vi "Obtain Request Events.vi"(8 "error in":errorcluster, 10 "Create New? (F)":bool, 11 "Module ID":i32=-1) -> (0 "error out":errorcluster, 2 "Function Generator Request Events":T1)   [LabVIEW 2026, in "Function Generator.lvlib"]
doc: "This VI Obtains/Creates the Requests events that will be used for other modules to communicate with the module that owns this VI. These Requests events will be accessed only via Public API methods for this module.\n\n<b>NOTE</b>: The contents of this VI are automatically generated and modified by the <b>Tools > DQMH Consortium > DQMH</b> utilities. Consider using those utilities instead of making your own modifications to this VI.\n_____\nBased on DQMH Dev Tools: Project Template 7.1.2.1547."
uses:
  Function Generator.lvlib
  Request Events--cluster.ctl
  Stop Argument--cluster.ctl
  Show Panel Argument--cluster.ctl
  Hide Panel Argument--cluster.ctl
  Show Diagram Argument--cluster.ctl
  Get Module Execution Status Argument--cluster.ctl
  Set Signal Type Argument--cluster.ctl
  Set Signal Parameters Argument--cluster.ctl
  Start Argument--cluster.ctl
  Local Instance Request Events--cluster.ctl
  Wake Up HL Argument--cluster.ctl
  Stop FGEN Argument--cluster.ctl
  Local Instance Events SEQ/Local Instance Events SEQ.lvlib
panel:
  # "NOTE: The contents of this VI are automatically generated and modified by the Tools > DQMH Consortium > DQMH utilities. Consider using those utilities instead of making your own modifications to this VI."
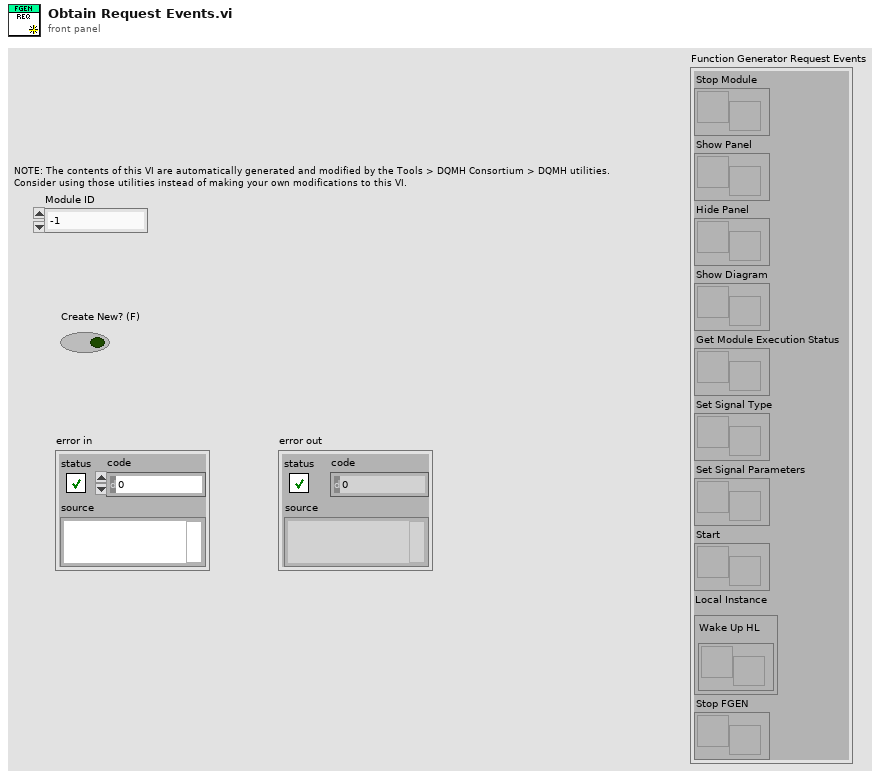
[diagram p1: front panel]
types:
  T1 = typedef "Function Generator.lvlib/Request Events--cluster.ctl" = cluster{"Stop Module":refnum<user-event>, "Show Panel":refnum<user-event>, "Hide Panel":refnum<user-event>, "Show Diagram":refnum<user-event>, "Get Module Execution Status":refnum<user-event>, "Set Signal Type":refnum<user-event>, "Set Signal Parameters":refnum<user-event>, "Start":refnum<user-event>, "Local Instance":T2, "Stop FGEN":refnum<user-event>}
  T2 = typedef "Function Generator.lvlib/Local Instance Request Events--cluster.ctl" = cluster{"Wake Up HL":refnum<user-event>}
  T3 = typedef "Function Generator.lvlib/Stop FGEN Argument--cluster.ctl" = cluster{"Module ID":i32, "Boolean":bool}
  T4 = typedef "Function Generator.lvlib/Start Argument--cluster.ctl" = cluster{"Module ID":i32, "Boolean":bool}
  T5 = typedef "Function Generator.lvlib/Set Signal Parameters Argument--cluster.ctl" = cluster{"Module ID":i32, "amplitude":dbl, "phase":dbl, "frequency":dbl, "offset":dbl}
  T6 = typedef "Function Generator.lvlib/Set Signal Type Argument--cluster.ctl" = cluster{"Module ID":i32, "signal type":enum16{"Sine Wave", "Triangle Wave", "Square Wave", "Sawtooth Wave"}}
  T7 = typedef "Function Generator.lvlib/Get Module Execution Status Argument--cluster.ctl" = cluster{"Module ID":i32, "Running?":bool}
  T8 = typedef "Function Generator.lvlib/Show Diagram Argument--cluster.ctl" = cluster{"Module ID":i32, "Debug?":bool}
  T9 = typedef "Function Generator.lvlib/Show Panel Argument--cluster.ctl" = cluster{"Module ID":i32, "Show Panel?":bool}
  T10 = typedef "Function Generator.lvlib/Hide Panel Argument--cluster.ctl" = cluster{"Module ID":i32, "Hide Panel?":bool}
  T11 = typedef "Function Generator.lvlib/Stop Argument--cluster.ctl" = cluster{"Module ID":i32, "Origin":string, "Exit via Stop Module Req?":bool, "Wait for Module to stop?":bool}
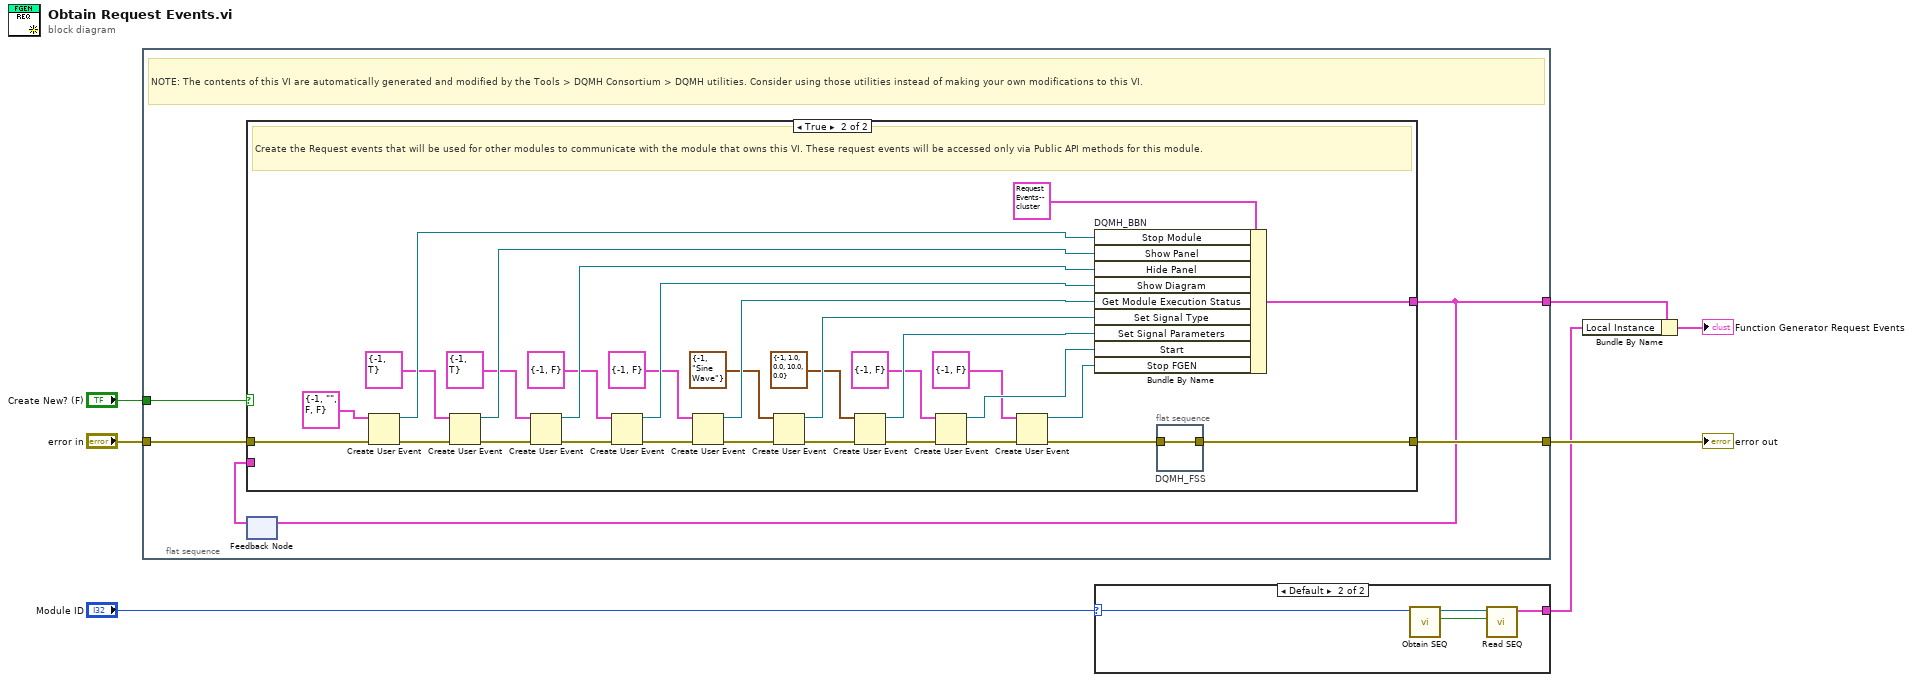
[diagram p0: block diagram]
diagram:
  n1 = flat-sequence {
    tunnel: [w12] -> w7
    tunnel: "error in" -> [w11]
    tunnel: [w9] -> w3
    tunnel: "Create New? (F)" -> [w8]
    frame #0 {
      # "NOTE: The contents of this VI are automatically generated and modified by the Tools > DQMH Consortium > DQMH utilities. Consider using those utilities instead of making your own modifications to this VI."
      n2 = feedback #1() -> (w10:T1)  [unwired: 1 in]
      n3 = case shown="True" w8 {
        tunnel: [w13 w33] -> w12
        tunnel: w11 -> [w13 w45]
        tunnel: [w14 w42] -> w9
        tunnel: w10 -> [w14 _]
        frame False {
        }
        frame True {
          # "Create the Request events that will be used for other modules to communicate with the module that owns this VI. These request events will be accessed only via Public API methods for this module."
          n4 = Create User Event(user event datatype=T11 {"Module ID"=-1, "Origin"="", "Exit via Stop Module Req?"=FALSE, "Wait for Module to stop?"=FALSE} ("Stop Argument"), error in=w45) -> (user event=w43:refnum<user-event>, error out=w40:errorcluster)
          n5 = Create User Event(user event datatype=T9 {"Module ID"=-1, "Show Panel?"=TRUE} ("Show Panel Argument"), error in=w40) -> (user event=w39:refnum<user-event>, error out=w37:errorcluster)
          n6 = Create User Event(user event datatype=T10 {"Module ID"=-1, "Hide Panel?"=TRUE} ("Hide Panel"), error in=w37) -> (user event=w36:refnum<user-event>, error out=w35:errorcluster)
          n7 = Create User Event(user event datatype=T8 {"Module ID"=-1, "Debug?"=FALSE} ("Show Diagram Argument"), error in=w35) -> (user event=w31:refnum<user-event>, error out=w32:errorcluster)
          n8 = Create User Event(user event datatype=T7 {"Module ID"=-1, "Running?"=FALSE} ("Get Module Execution Status Argument"), error in=w32) -> (user event=w28:refnum<user-event>, error out=w29:errorcluster)
          n9 = Create User Event(user event datatype=T6 {"Module ID"=-1, "signal type"=enum."Sine Wave"} ("Set Signal Type Argument"), error in=w29) -> (user event=w25:refnum<user-event>, error out=w26:errorcluster)
          n10 = Create User Event(user event datatype=T5 {"Module ID"=-1, "amplitude"=1.0, "phase"=0.0, "frequency"=10.0, "offset"=0.0} ("Set Signal Parameters Argument"), error in=w26) -> (user event=w22:refnum<user-event>, error out=w23:errorcluster)
          n11 = Create User Event(user event datatype=T4 {"Module ID"=-1, "Boolean"=FALSE} ("Start Argument"), error in=w23) -> (user event=w19:refnum<user-event>, error out=w20:errorcluster)
          n12 = Create User Event(user event datatype=T3 {"Module ID"=-1, "Boolean"=FALSE} ("Stop FGEN Argument"), error in=w20) -> (user event=w16:refnum<user-event>, error out=w17:errorcluster)
          n13 = Bundle By Name "DQMH_BBN"(cluster=T1 {"Stop Module"=refnum, "Show Panel"=refnum, "Hide Panel"=refnum, "Show Diagram"=refnum, "Get Module Execution Status"=refnum, "Set Signal Type"=refnum, "Set Signal Parameters"=refnum, "Start"=refnum, "Local Instance"={"Wake Up HL"=refnum}, "Stop FGEN"=refnum} ("output cluster"), "Stop Module"=w43, "Show Panel"=w39, "Hide Panel"=w36, "Show Diagram"=w31, "Get Module Execution Status"=w28, "Set Signal Type"=w25, "Set Signal Parameters"=w22, "Start"=w19, "Stop FGEN"=w16) -> (w42:T1)
          n14 = flat-sequence "DQMH_FSS" {
            tunnel: w17 -> [w46]
            tunnel: [w46] -> w33
            frame #0 {
            }
          }
        }
      }
      n15 = feedback-in #1(w9) -> ()
    }
  }
  n16 = case shown="Default" "Module ID" {
    selector: "Module ID" -> [_ w48]
    tunnel: [_ w47] -> w2
    frame -1 {
    }
    frame Default {
      n17 = call "Obtain SEQ.vi"("Module ID"=w48) -> ("Created New?"=w49:bool, "Local Instance Event SEQ"=w50:refnum<queue>)  [unwired: 8 in, 1 out]
      n18 = call "Read SEQ.vi"("Created New?"=w49, "Local Instance Event SEQ"=w50) -> ("Local Instance Request Events"=w47:T2)  [unwired: 8 in, 1 out]
    }
  }
  n19 = Bundle By Name(cluster=w3, "Local Instance"=w2) -> (→"Function Generator Request Events":T1)
  "error out" <- w7
